vi "Main.vi"() -> ()   [LabVIEW 2026]
uses:
  Typedefs/Test Config.ctl
  Typedefs/Station State.ctl
  Typedefs/Measurement.ctl
  Typedefs/Log Message.ctl
  Typedefs/Log Message Type.ctl
  Typedefs/Chiller Action.ctl
  <vilib>/drjdpowell/SQLite Library/SQL Connection/Connection.lvclass/Connection.ctl
  <vilib>/drjdpowell/SQLite Library/SQL Connection/Execute SQL (No results).vi
  <vilib>/drjdpowell/SQLite Library/SQL Connection/Connection.lvclass
  <vilib>/Analysis/NI_AALPro.lvlib
  <vilib>/drjdpowell/SQLite Library/SQLite.lvlib
panel:
  out "Runs Synced":i32
  out "# elements in queue":i32
  out "Abort Reason":string
  out "Result":string
  out "L-I Curve":cluster{dbl[], dbl[]}(graph)
  out "Power (W)":dbl
  out "Current (A)":dbl
  out "Chiller Temp (C)":dbl
  out "State":T1
  in  "Interlock OK":bool=TRUE
  in  "Quit":bool
  in  "Run Batch":bool
  in  "Abort":bool
  in  "Start":bool
  in  "Test Config":T2={"Setpoint (C)"=25.0, "Serial Number"="LD-0001", "I Start (A)"=0.0, "I Stop (A)"=6.0, "I Step (A)"=0.1, "Ith Max (A)"=0.6, "Slope Min (W/A)"=0.9, "Stabilize Tol (C)"=0.2, "Stabilize Timeout (s)"=300.0, "Over-Temp Limit (C)"=40.0, "Operator"="mahmut", "Fit I Max (A)"=3.0, "Fit P Min (W)"=0.1}
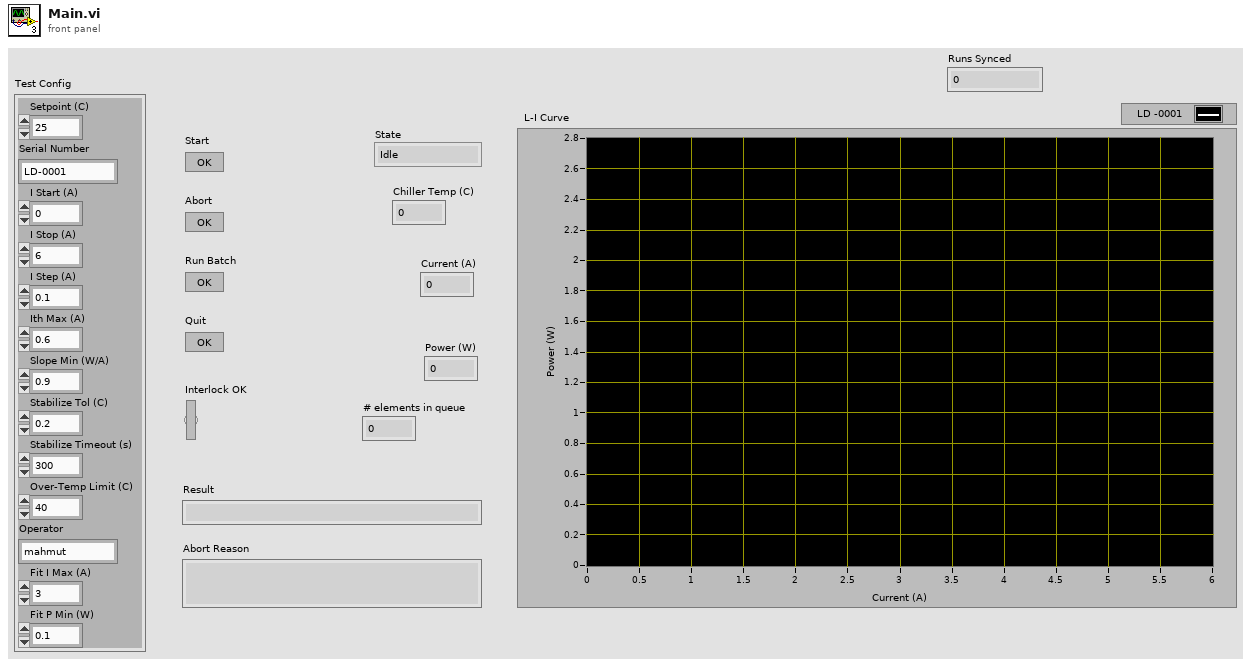
[diagram p1: front panel]
types:
  T1 = typedef "Station State.ctl" = enum16{"Idle", "Initialize", "Chiller Stabilize", "Current Ramp", "Measure", "Evaluate", "Log", "Report", "Safe Shutdown"}
  T2 = typedef "Test Config.ctl" = cluster{"Setpoint (C)":dbl, "Serial Number":string, "I Start (A)":dbl, "I Stop (A)":dbl, "I Step (A)":dbl, "Ith Max (A)":dbl, "Slope Min (W/A)":dbl, "Stabilize Tol (C)":dbl, "Stabilize Timeout (s)":dbl, "Over-Temp Limit (C)":dbl, "Operator":string, "Fit I Max (A)":dbl, "Fit P Min (W)":dbl}
  T3 = typedef "Log Message.ctl" = cluster{"Type":T4, "Serial Number":string, "Measurement":T5, "Pass":bool, "Ith (A)":dbl, "Slope (W/A)":dbl, "Reason":string}
  T4 = typedef "Log Message Type.ctl" = enum16{"Run Start", "Measurement", "Run End", "Stop"}
  T5 = typedef "Measurement.ctl" = cluster{"Current (A)":dbl, "Power (W)":dbl, "Temp (C)":dbl, "t (s)":dbl}
  T6 = enum16{"open", "replace", "create", "open or create", "replace or create", "replace or create with confirmation"}
  T7 = cluster{"Last INSERT RowID":i64, i32, "Current (A)":dbl, "Power (W)":dbl, "Temp (C)":dbl, "t (s)":dbl}
  T8 = cluster{string, "Ith (A)":dbl, "Slope (W/A)":dbl, "Variant":variant, "Reason":string, "Last INSERT RowID":i64}
  T9 = typedef "Chiller Action.ctl" = enum16{"Init", "Set Setpoint", "Step", "Read"}
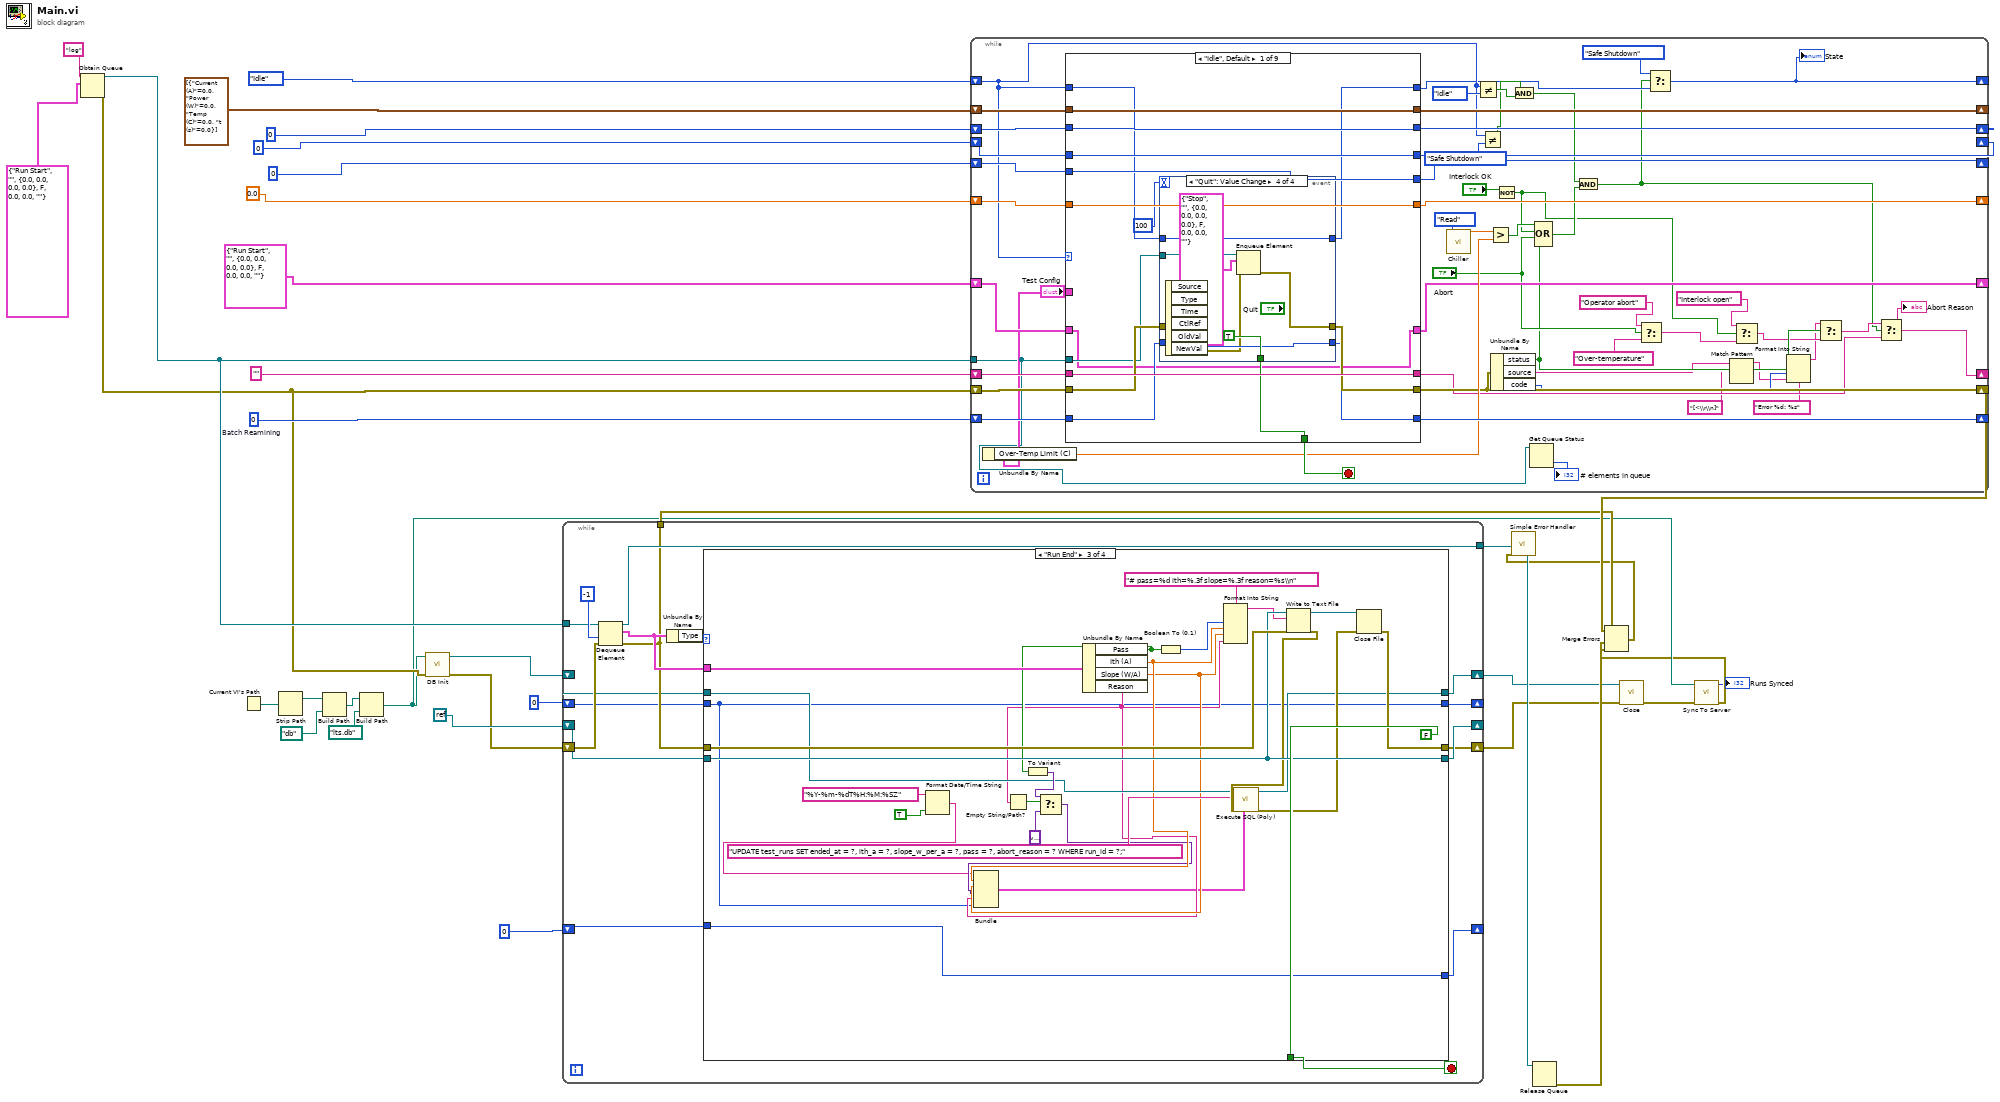
[diagram p0: block diagram]
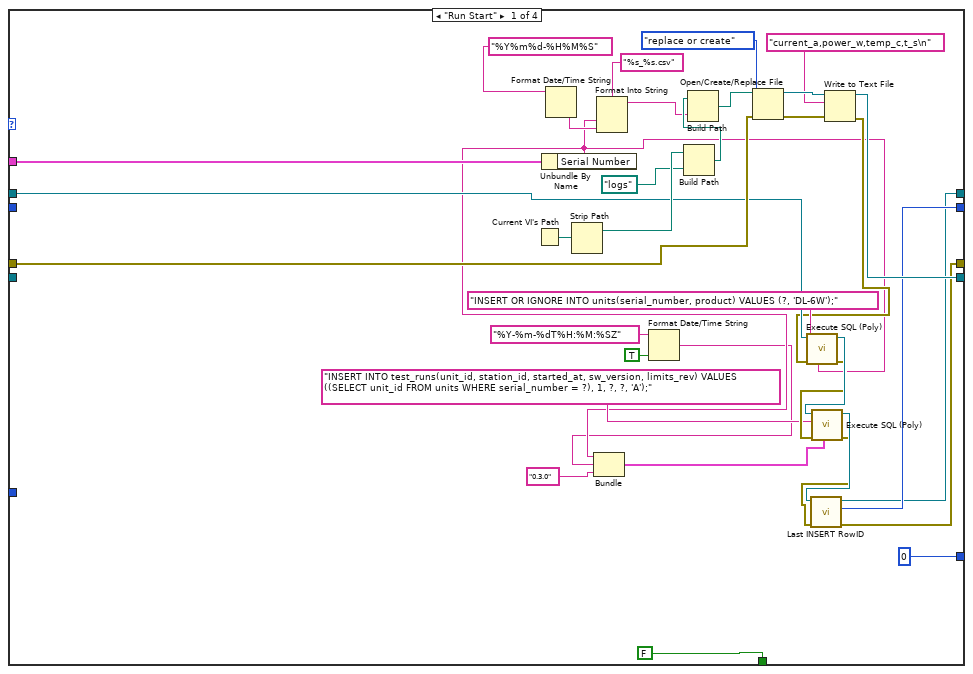
[diagram p2: hidden frame]
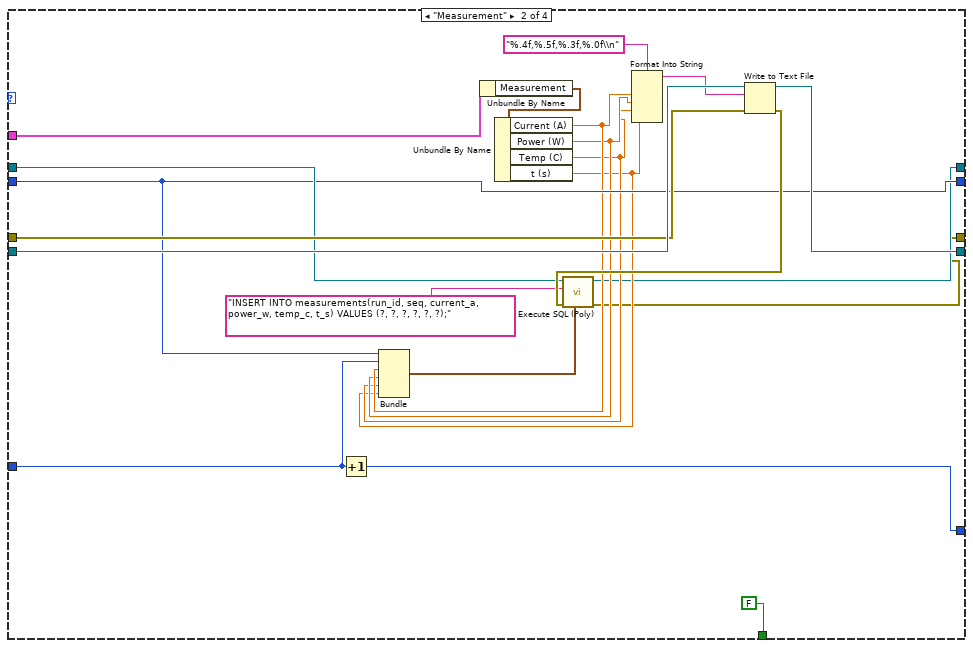
[diagram p3: hidden frame]
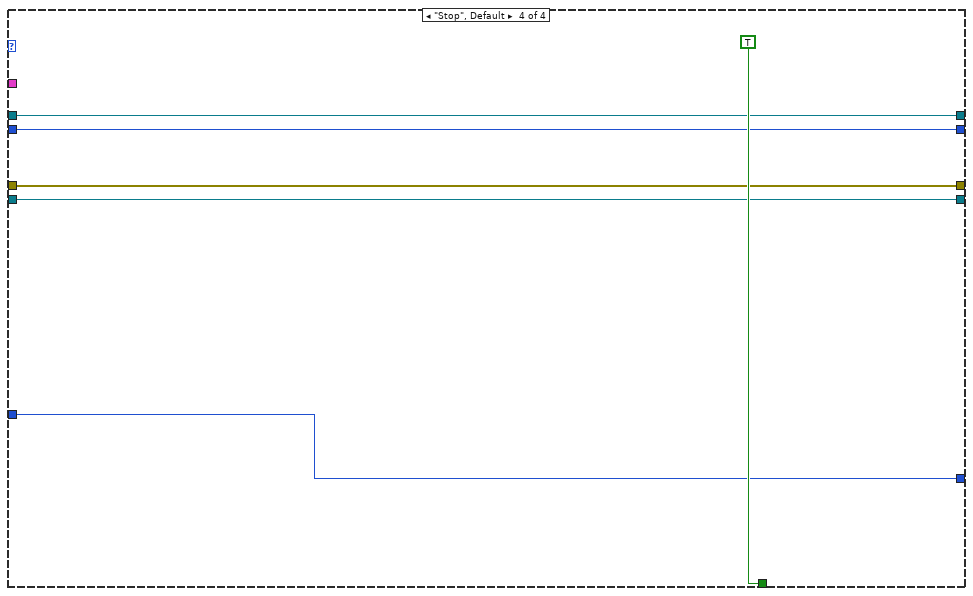
[diagram p4: hidden frame]
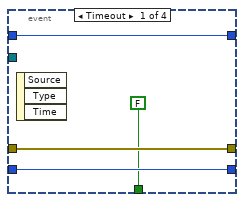
[diagram p5: hidden frame]
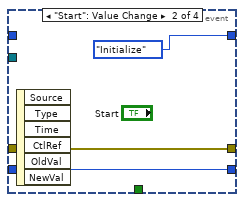
[diagram p6: hidden frame]
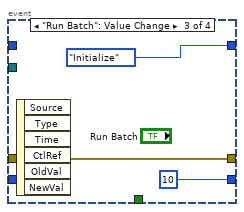
[diagram p7: hidden frame]
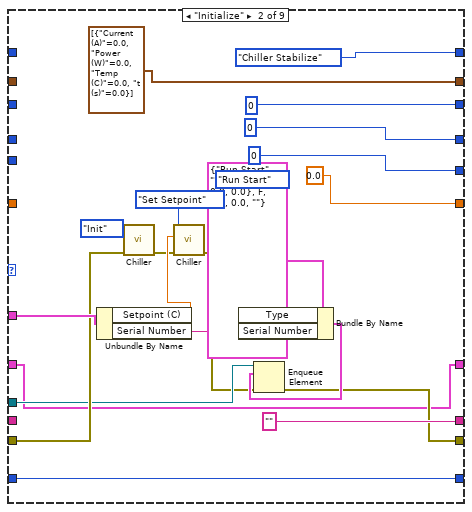
[diagram p8: hidden frame]
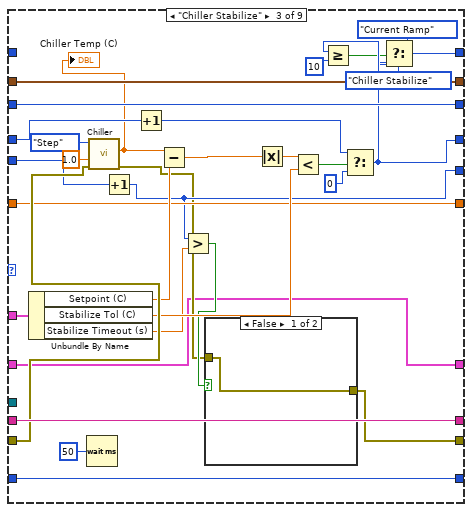
[diagram p9: hidden frame]
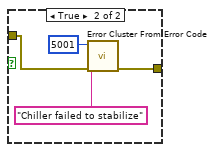
[diagram p10: hidden frame]
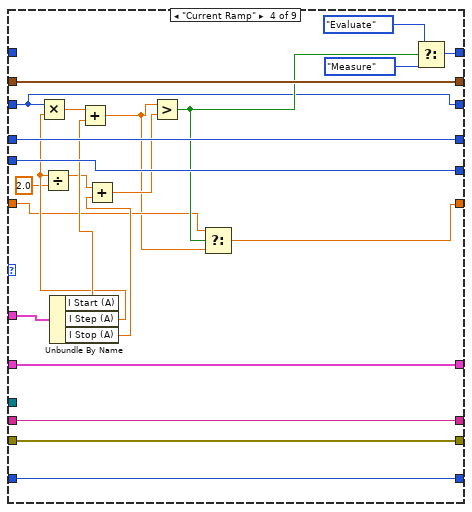
[diagram p11: hidden frame]
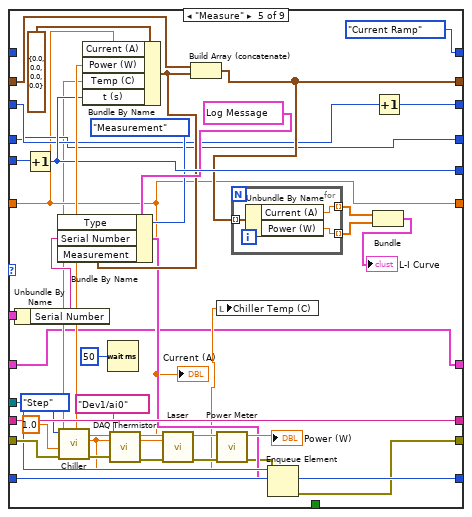
[diagram p12: hidden frame]
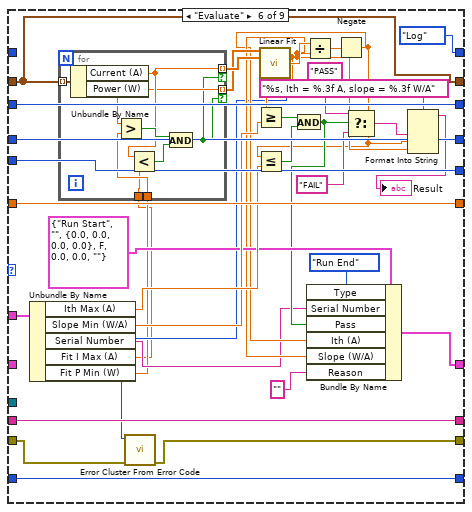
[diagram p13: hidden frame]
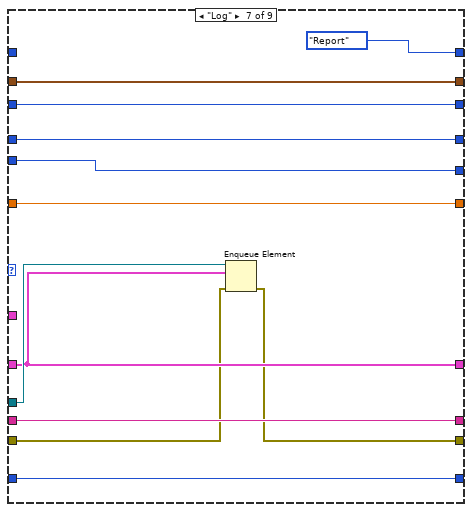
[diagram p14: hidden frame]
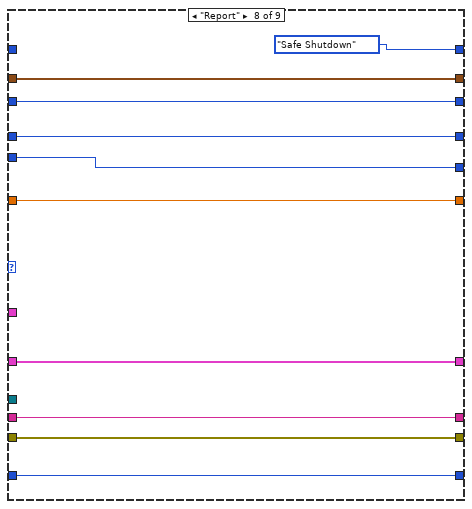
[diagram p15: hidden frame]
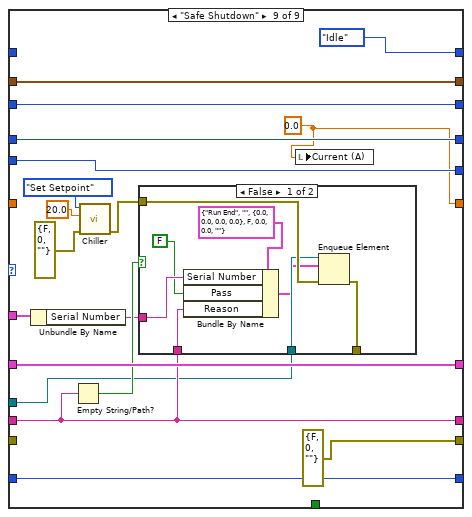
[diagram p16: hidden frame]
diagram:
  w19 = 0  # Batch Reamining
  n1 = Obtain Queue(name (unnamed)="log", element data type=T3 {"Type"=enum."Run Start", "Serial Number"="", "Measurement"={"Current (A)"=0.0, "Power (W)"=0.0, "Temp (C)"=0.0, "t (s)"=0.0}, "Pass"=FALSE, "Ith (A)"=0.0, "Slope (W/A)"=0.0, "Reason"=""} ("Log Message")) -> (queue out=w25:refnum<queue>, error out=w11:errorcluster)  [unwired: 3 in, 1 out]
  n2 = Current VI's Path() -> (path=w16:path)
  n3 = Strip Path(path=w16) -> (stripped path=w15:path)  [unwired: 1 out]
  n4 = Build Path(base path=w15, name or relative path=path "db") -> (appended path=w13:path)
  n5 = Build Path(base path=w13, name or relative path=path "lts.db") -> (appended path=w4:path)
  n6 = call "DB Init.vi"("error in (no error)"=w11, "DB Path"=w4) -> ("error out"=w10:errorcluster, "Connection"=w9:refnum<class "Connection.lvclass">)  [unwired: 8 in]
  n7 = while {
    tunnel: w25 -> [w50]
    tunnel: [w44] -> w23
    tunnel: [w46] -> w21
    shift-right: [w42] -> _
    shift-left: refnum<k0> refnum -> [w43]
    shift-right: [w39] -> w7
    shift-left: w9 -> [w41]
    shift-right: [w37] -> _
    shift-left: i64 0 -> [w40]
    shift-right: [w38] -> w6
    shift-left: w10 -> [w47]
    shift-right: [w35] -> _
    shift-left: 0 -> [w36]
    stop <- w48 stop-if-true
    n8 = Dequeue Element(queue=w50, timeout in ms (-1)=-1, error in (no error)=w47) -> (queue out=w46:refnum<queue>, element=w45:T3, error out=w44:errorcluster)  [unwired: 1 out]
    n9 = Unbundle By Name "Unbundle By Name"(w45) -> ("Type"=w49:T4)
    n10 = case shown="\"Run End\"" w49 {
      tunnel: [FALSE FALSE FALSE TRUE] -> w48
      tunnel: w45 -> [w85 w106 w134 _]
      tunnel: w44 -> [w80 w101 w131 w139]
      tunnel: w43 -> [_ w103 w129 w140]
      tunnel: [w53 w87 w130 w139] -> w38
      tunnel: [w77 w102 w129 w140] -> w42
      tunnel: w41 -> [w69 w97 w118 w138]
      tunnel: [w54 w88 w117 w138] -> w39
      tunnel: w40 -> [_ w95 w108 w137]
      tunnel: [w55 w95 w108 w137] -> w37
      tunnel: w36 -> [_ w94 w111 w136]
      tunnel: [0 w99 w111 w136] -> w35
      frame "Run Start" {
        n11 = Current VI's Path() -> (path=w82:path)
        n12 = Unbundle By Name(w85) -> ("Serial Number"=w61:string)
        n13 = Format Date/Time String(time format string (%c)="%Y%m%d-%H%M%S") -> (date/time string=w75:string)  [unwired: 2 in]
        n14 = Strip Path(path=w82) -> (stripped path=w74:path)  [unwired: 1 out]
        n15 = Format Into String "Format Into String"(format string="%s_%s.csv", w61, w75) -> (resulting string=w71:string)  [unwired: 2 in, 1 out]
        n16 = Format Date/Time String(time format string (%c)="%Y-%m-%dT%H:%M:%SZ", UTC format=TRUE) -> (date/time string=w60:string)  [unwired: 1 in]
        n17 = Bundle("Serial Number"=w61, w60, "0.3.0") -> (w58:cluster{"Serial Number":string, string, string})  [unwired: 1 in]
        n18 = Build Path(base path=w74, name or relative path=path "logs") -> (appended path=w72:path)
        n19 = Build Path(base path=w72, name or relative path=w71) -> (appended path=w81:path)
        n20 = Open/Create/Replace File(file path (use dialog)=w81, error in=w80, operation (0:open)=T6."replace or create") -> (refnum out=w78:refnum<file>, error out=w79:errorcluster)  [unwired: 3 in, 1 out]
        n21 = Write to Text File(file (use dialog)=w78, text="current_a,power_w,temp_c,t_s\n", error in=w79) -> (refnum out=w77:refnum<file>, error out=w67:errorcluster)  [unwired: 1 in, 1 out]
        n22 = call-poly <vilib>:"Execute SQL (Poly).vi"("Parameter(s)"=w61, "error in (no error)"=w67, "SQL"="INSERT OR IGNORE INTO units(serial_number, product) VALUES (?, 'DL-6W');", "SQLite Connection in"=w69) -> ("error out"=w63:errorcluster, "SQLite Connection"=w64:refnum<class "Connection.lvclass">)  [unwired: 6 in]
        n23 = call-poly <vilib>:"Execute SQL (Poly).vi"("Parameter(s)"=w58, "error in (no error)"=w63, "SQL"="INSERT INTO test_runs(unit_id, station_id, started_at, sw_version, limits_rev) VALUES ((SELECT unit_id FROM units WHERE serial_number = ?), 1, ?, ?, 'A');", "SQLite Connection in"=w64) -> ("error out"=w56:errorcluster, "SQLite Connection"=w57:refnum<class "Connection.lvclass">)  [unwired: 6 in]
        n24 = call <vilib>:"Last INSERT RowID.vi"("error in (no error)"=w56, "SQLite Connection in"=w57) -> ("error out"=w53:errorcluster, "Last INSERT RowID"=w55:i64, "SQLite Connection"=w54:refnum<class "Connection.lvclass">)  [unwired: 7 in]
      }
      frame "Measurement" {
        n25 = Increment(x=w94) -> (x+1=w99:i32)
        n26 = Unbundle By Name(w106) -> ("Measurement"=w105:T5)
        n27 = Unbundle By Name(w105) -> ("Current (A)"=w93:dbl, "Power (W)"=w92:dbl, "Temp (C)"=w91:dbl, "t (s)"=w90:dbl)
        n28 = Bundle("Last INSERT RowID"=w95, w94, "Current (A)"=w93, "Power (W)"=w92, "Temp (C)"=w91, "t (s)"=w90) -> (w89:T7)  [unwired: 1 in]
        n29 = Format Into String(format string="%.4f,%.5f,%.3f,%.0f\\n", w93, w92, w91, w90) -> (resulting string=w100:string)  [unwired: 2 in, 1 out]
        n30 = Write to Text File(file (use dialog)=w103, text=w100, error in=w101) -> (refnum out=w102:refnum<file>, error out=w98:errorcluster)  [unwired: 1 in, 1 out]
        n31 = call-poly <vilib>:"Execute SQL (Poly).vi"("Parameter(s)"=w89, "error in (no error)"=w98, "SQL"="INSERT INTO measurements(run_id, seq, current_a, power_w, temp_c, t_s) VALUES (?, ?, ?, ?, ?, ?);", "SQLite Connection in"=w97) -> ("error out"=w87:errorcluster, "SQLite Connection"=w88:refnum<class "Connection.lvclass">)  [unwired: 6 in]
      }
      frame "Run End" {
        n32 = Format Date/Time String(time format string (%c)="%Y-%m-%dT%H:%M:%SZ", UTC format=TRUE) -> (date/time string=w109:string)  [unwired: 1 in]
        n33 = Unbundle By Name(w134) -> ("Pass"=w124:bool, "Ith (A)"=w115:dbl, "Slope (W/A)"=w114:dbl, "Reason"=w112:string)
        n34 = Empty String/Path?(string/path=w112) -> (empty?=w123:bool)
        n35 = To Variant(anything=w124) -> (Variant=w122:variant)
        n36 = Select(t=w122, s=w123, f=variant) -> (s? t:f=w113:variant)
        n37 = Bundle(w109, "Ith (A)"=w115, "Slope (W/A)"=w114, "Variant"=w113, "Reason"=w112, "Last INSERT RowID"=w108) -> (w110:T8)  [unwired: 1 in]
        n38 = Boolean To (0,1)(Boolean=w124) -> (0, 1=w132:i16)
        n39 = Format Into String(format string="# pass=%d ith=%.3f slope=%.3f reason=%s\\n", w132, w115, w114, w112) -> (resulting string=w127:string)  [unwired: 2 in, 1 out]
        n40 = Write to Text File(file (use dialog)=w129, text=w127, error in=w131) -> (refnum out=w128:refnum<file>, error out=w120:errorcluster)  [unwired: 1 in, 1 out]
        n41 = call-poly <vilib>:"Execute SQL (Poly).vi"("Parameter(s)"=w110, "error in (no error)"=w120, "SQL"="UPDATE test_runs SET ended_at = ?, ith_a = ?, slope_w_per_a = ?, pass = ?, abort_reason = ? WHERE run_id = ?;", "SQLite Connection in"=w118) -> ("error out"=w119:errorcluster, "SQLite Connection"=w117:refnum<class "Connection.lvclass">)  [unwired: 6 in]
        n42 = Close File(refnum=w128, error in=w119) -> (error out=w130:errorcluster)  [unwired: 1 out]
      }
      frame "Stop", Default {
      }
    }
  }
  n43 = while {
    shift-right: [w151] -> _
    shift-left: Station_State."Idle" ("Enum") -> [w171]
    shift-right: [w194] -> _
    shift-left: T5[] [{"Current (A)"=0.0, "Power (W)"=0.0, "Temp (C)"=0.0, "t (s)"=0.0}] -> [w195]
    shift-right: [w192] -> _
    shift-left: 0 -> [w193]
    shift-right: [w190] -> _
    shift-left: 0 -> [w191]
    shift-right: [w188] -> _
    shift-left: 0 -> [w189]
    shift-right: [w186] -> _
    shift-left: 0.0 -> [w187]
    shift-right: [w150] -> _
    shift-left: "" -> [w185]
    shift-right: [w175] -> w24
    shift-left: w11 -> [w184]
    tunnel: w25 -> [w149]
    shift-right: [w181] -> _
    shift-left: w19 -> [w182]
    shift-right: [w165] -> _
    shift-left: T3 {"Type"=enum."Run Start", "Serial Number"="", "Measurement"={"Current (A)"=0.0, "Power (W)"=0.0, "Temp (C)"=0.0, "t (s)"=0.0}, "Pass"=FALSE, "Ith (A)"=0.0, "Slope (W/A)"=0.0, "Reason"=""} ("Log Message") -> [w180]
    stop <- w183 stop-if-true
    n44 = Unbundle By Name("Test Config") -> ("Over-Temp Limit (C)"=w177:dbl)
    n45 = case shown="\"Idle\", Default" w171 {
      tunnel: w171 -> [w205 _ _ _ _ _ _ _ _]
      tunnel: [w204 Station_State."Chiller Stabilize" ("Enum") w259 w295 Station_State."Current Ramp" ("Enum") Station_State."Log" ("Enum") Station_State."Report" ("Enum") Station_State."Safe Shutdown" ("Enum") Station_State."Idle" ("Enum")] -> w164
      tunnel: [w211 T5[] [{"Current (A)"=0.0, "Power (W)"=0.0, "Temp (C)"=0.0, "t (s)"=0.0}] w264 w310 w321 w378 w404 w414 w432] -> w194
      tunnel: w195 -> [w211 _ w264 w310 w331 w378 w404 w414 w432]
      tunnel: [w210 0 w282 w289 w316 w384 w403 w413 w431] -> w192
      tunnel: w193 -> [w210 _ w282 w289 w317 w384 w403 w413 w431]
      tunnel: [w209 0 w263 w309 w314 w383 w402 w412 w430] -> w190
      tunnel: w191 -> [w209 _ w270 w309 w314 w383 w402 w412 w430]
      tunnel: [w208 0 w258 w308 w332 w382 w401 w411 w429] -> w188
      tunnel: w189 -> [w208 _ w266 w308 w333 w382 w401 w411 w429]
      tunnel: [w207 0.0 w268 w290 w313 w381 w400 w410 w422] -> w186
      tunnel: w187 -> [w207 _ w268 w292 w313 w381 w400 w410 _]
      tunnel: [w206 "" w281 w307 w346 w356 w399 w409 w416] -> w153
      tunnel: w185 -> [w206 _ w281 w307 w346 w356 w399 w409 w416]
      tunnel: [w202 w230 w253 w306 w322 w353 w393 w408 errorcluster {"status"=FALSE, "code"=0, "source"=""} ("error constant")] -> w175
      tunnel: w184 -> [w203 w244 w276 w306 w344 w354 w394 w408 _]
      tunnel: [w199 _ _ _ _ _ _ _ _] -> w183
      tunnel: w182 -> [w201 w250 w280 w305 w341 w380 w398 w407 w428]
      tunnel: [w200 w250 w280 w305 w341 w380 w398 w407 w428] -> w181
      tunnel: w149 -> [w197 w233 _ _ w325 _ w396 _ w415]
      tunnel: "Test Config" -> [_ w248 w279 w304 w328 w373 _ _ w418]
      tunnel: w180 -> [w196 w229 w251 w288 w311 _ w395 w405 w426]
      tunnel: [w196 w229 w251 w288 w311 w360 w395 w405 w426] -> w165
      frame "Idle", Default {
        n46 = event shown="[3] \"Quit\": Value Change" {
          selector: _ -> [_ _ _ _]
          dyn-events: _ -> [_ _ _ _]
          timeout: 100 -> [_ _ _ _]
          tunnel: w205 -> [w215 _ _ w228]
          tunnel: [w215 Station_State."Initialize" ("Enum") Station_State."Initialize" ("Enum") w228] -> w204
          tunnel: w203 -> [w214 w217 w219 w224]
          tunnel: [w214 w217 w219 w223] -> w202
          tunnel: w201 -> [w213 w218 _ w226]
          tunnel: [w213 w218 10 ("Batch Reamining") w226] -> w200
          tunnel: [FALSE _ _ TRUE] -> w199
          tunnel: w197 -> [_ _ _ w225]
          event Timeout {
            n47 = event-data() -> ()  [unwired: 1 in, 3 out]
          }
          event "Start": Value Change {
            n48 = event-data() -> ()  [unwired: 1 in, 6 out]
          }
          event "Run Batch": Value Change {
            n49 = event-data() -> ()  [unwired: 1 in, 6 out]
          }
          event "Quit": Value Change {
            n50 = event-data() -> ()  [unwired: 1 in, 6 out]
            n51 = Enqueue Element(queue=w225, element=T3 {"Type"=enum."Stop", "Serial Number"="", "Measurement"={"Current (A)"=0.0, "Power (W)"=0.0, "Temp (C)"=0.0, "t (s)"=0.0}, "Pass"=FALSE, "Ith (A)"=0.0, "Slope (W/A)"=0.0, "Reason"=""} ("Log Message"), error in (no error)=w224) -> (error out=w223:errorcluster)  [unwired: 1 in, 2 out]
          }
        }
      }
      frame "Initialize" {
        n52 = Unbundle By Name(w248) -> ("Setpoint (C)"=w245:dbl, "Serial Number"=w234:string)
        n53 = call "Chiller.vi"("error in (no error)"=w244, "Action"=Chiller_Action."Init") -> ("error out"=w243:errorcluster)  [unwired: 5 in, 2 out]
        n54 = call "Chiller.vi"("error in (no error)"=w243, "Setpoint (C)"=w245, "Action"=Chiller_Action."Set Setpoint") -> ("error out"=w231:errorcluster)  [unwired: 4 in, 2 out]
        n55 = Bundle By Name(cluster=T3 {"Type"=enum."Run Start", "Serial Number"="", "Measurement"={"Current (A)"=0.0, "Power (W)"=0.0, "Temp (C)"=0.0, "t (s)"=0.0}, "Pass"=FALSE, "Ith (A)"=0.0, "Slope (W/A)"=0.0, "Reason"=""} ("Log Message"), "Type"=Log_Message_Type."Run Start", "Serial Number"=w234) -> (w232:T3)
        n56 = Enqueue Element(queue=w233, element=w232, error in (no error)=w231) -> (error out=w230:errorcluster)  [unwired: 1 in, 2 out]
      }
      frame "Chiller Stabilize" {
        n57 = Unbundle By Name(w279) -> ("Setpoint (C)"=w275:dbl, "Stabilize Tol (C)"=w272:dbl, "Stabilize Timeout (s)"=w257:dbl)
        n58 = Wait (ms)(milliseconds to wait=u32 50) -> ()  [unwired: 1 out]
        n59 = call "Chiller.vi"("error in (no error)"=w276, "dt (s)"=1.0, "Action"=Chiller_Action."Step") -> ("error out"=w254:errorcluster, "Temp (C)"=w255:dbl)  [unwired: 4 in, 1 out]
        "Chiller Temp (C)" <- w255
        n60 = Increment(x=w266) -> (x+1=w258:i32)
        n61 = Increment(x=w270) -> (x+1=w269:i32)
        n62 = Subtract(x=w255, y=w275) -> (x-y=w274:dbl)
        n63 = Greater?(x=w258, y=w257) -> (0:w256:bool)
        n64 = case shown="False" w256 {
          tunnel: w254 -> [w283 w285]
          tunnel: [w283 w284] -> w253
          frame False {
          }
          frame True {
            n65 = call <vilib>:"Error Cluster From Error Code.vi"("error in (no error)"=w285, "error message (\"\")"="Chiller failed to stabilize" ("error message (\"\")"), "error code (0)"=5001) -> ("error out"=w284:errorcluster)  [unwired: 6 in]
          }
        }
        n66 = Absolute Value(x=w274) -> (abs(x)=w273:dbl)
        n67 = Less?(x=w273, y=w272) -> (x < y?=w271:bool)
        n68 = Select(t=w269, s=w271, f=0) -> (s? t:f=w263:i32)
        n69 = Greater Or Equal?(x=w263, y=10) -> (x >= y?=w262:bool)
        n70 = Select(t=Station_State."Current Ramp" ("Enum"), s=w262, f=Station_State."Chiller Stabilize" ("Enum")) -> (s? t:f=w259:T1)
      }
      frame "Current Ramp" {
        n71 = Unbundle By Name(w304) -> ("I Start (A)"=w302:dbl, "I Step (A)"=w300:dbl, "I Stop (A)"=w301:dbl)
        n72 = Multiply(x=w289, y=w300) -> (x*y=w303:dbl)
        n73 = Divide(x=w300, y=2.0) -> (x/y=w298:dbl)
        n74 = Add(x=w303, y=w302) -> (x+y=w291:dbl)
        n75 = Add(x=w298, y=w301) -> (x+y=w299:dbl)
        n76 = Greater?(x=w291, y=w299) -> (0:w293:bool)
        n77 = Select(t=w292, s=w293, f=w291) -> (s? t:f=w290:dbl)
        n78 = Select(t=Station_State."Evaluate" ("Enum"), s=w293, f=Station_State."Measure" ("Enum")) -> (s? t:f=w295:T1)
      }
      frame "Measure" {
        n79 = Unbundle By Name(w328) -> ("Serial Number"=w327:string)
        n80 = Increment(x=w333) -> (x+1=w332:i32)
        n81 = call "Chiller.vi"("error in (no error)"=w344, "dt (s)"=1.0, "Action"=Chiller_Action."Step") -> ("error out"=w339:errorcluster, "Temp (C)"=w312:dbl)  [unwired: 4 in, 1 out]
        n82 = Wait (ms)(milliseconds to wait=u32 50) -> ()  [unwired: 1 out]
        n83 = call "DAQ Thermistor.vi"("error in (no error)"=w339, "DAQmx Physical Channel"=tag "Dev1/ai0") -> ("error out"=w338:errorcluster)  [unwired: 7 in, 2 out]
        n84 = call "Laser.vi"("error in (no error)"=w338, "Temp (C)"=w312, "Current (A)"=w313) -> ("error out"=w337:errorcluster, "Power (W)"=w336:dbl)  [unwired: 6 in, 1 out]
        n85 = local write "Chiller Temp (C)"(w312) -> ()
        n86 = call "Power Meter.vi"("error in (no error)"=w337, "True Power (W)"=w336) -> ("error out"=w323:errorcluster, "Reading (W)"=w334:dbl)  [unwired: 8 in]
        "Power (W)" <- w334
        n87 = Bundle By Name(cluster=T5 {"Current (A)"=0.0, "Power (W)"=0.0, "Temp (C)"=0.0, "t (s)"=0.0} ("Cluster"), "Current (A)"=w313, "Power (W)"=w334, "Temp (C)"=w312, "t (s)"=w332) -> (w326:T5)
        n88 = Bundle By Name(cluster=T3 {"Type"=enum."Run Start", "Serial Number"="", "Measurement"={"Current (A)"=0.0, "Power (W)"=0.0, "Temp (C)"=0.0, "t (s)"=0.0}, "Pass"=FALSE, "Ith (A)"=0.0, "Slope (W/A)"=0.0, "Reason"=""} ("Log Message"), "Type"=Log_Message_Type."Measurement", "Serial Number"=w327, "Measurement"=w326) -> (w324:T3)
        n89 = Build Array (concatenate)(w331, w326) -> (w321:T5[])
        n90 = for {
          tunnel: w321 -> [w349] mode=indexing
          tunnel: [w348] -> w320 mode=indexing
          tunnel: [w347] -> w319 mode=indexing
          n91 = Unbundle By Name(w349) -> ("Current (A)"=w348:dbl, "Power (W)"=w347:dbl)
        }
        n92 = Enqueue Element(queue=w325, element=w324, error in (no error)=w323) -> (error out=w322:errorcluster)  [unwired: 1 in, 2 out]
        n93 = Bundle(w320, w319) -> (→"L-I Curve":cluster{dbl[], dbl[]})  [unwired: 1 in]
        n94 = Increment(x=w317) -> (x+1=w316:i32)
        "Current (A)" <- w313
      }
      frame "Evaluate" {
        n95 = Unbundle By Name(w373) -> ("Ith Max (A)"=w372:dbl, "Slope Min (W/A)"=w371:dbl, "Serial Number"=w352:string, "Fit I Max (A)"=w350:dbl, "Fit P Min (W)"=w351:dbl)
        n96 = for {
          tunnel: w378 -> [w392] mode=indexing
          tunnel: [w389] -> w377 mode=indexing if=w387
          tunnel: [w388] -> w376 mode=indexing if=w387
          tunnel: w351 -> [w386]
          tunnel: w350 -> [w385]
          n97 = Unbundle By Name(w392) -> ("Current (A)"=w389:dbl, "Power (W)"=w388:dbl)
          n98 = Greater?(x=w388, y=w386) -> (0:w391:bool)
          n99 = Less?(x=w389, y=w385) -> (x < y?=w390:bool)
          n100 = And(x=w391, y=w390) -> (x .and. y?=w387:bool)
        }
        n101 = call <vilib>:"Linear Fit.vi"("Y"=w376, "X"=w377) -> ("slope"=w358:dbl, "intercept"=w375:dbl, "error"=w355:i32)  [unwired: 9 in, 2 out]
        n102 = call <vilib>:"Error Cluster From Error Code.vi"("error in (no error)"=w354, "error code (0)"=w355) -> ("error out"=w353:errorcluster)  [unwired: 7 in]
        n103 = Greater Or Equal?(x=w358, y=w371) -> (x >= y?=w370:bool)
        n104 = Divide(x=w375, y=w358) -> (x/y=w374:dbl)
        n105 = Negate(x=w374) -> (-x=w357:dbl)
        n106 = Less Or Equal?(x=w357, y=w372) -> (x <= y?=w369:bool)
        n107 = And(x=w370, y=w369) -> (x .and. y?=w359:bool)
        n108 = Bundle By Name(cluster=T3 {"Type"=enum."Run Start", "Serial Number"="", "Measurement"={"Current (A)"=0.0, "Power (W)"=0.0, "Temp (C)"=0.0, "t (s)"=0.0}, "Pass"=FALSE, "Ith (A)"=0.0, "Slope (W/A)"=0.0, "Reason"=""} ("Log Message"), "Type"=Log_Message_Type."Run End", "Serial Number"=w352, "Pass"=w359, "Ith (A)"=w357, "Slope (W/A)"=w358, "Reason"="") -> (w360:T3)
        n109 = Select(t="PASS", s=w359, f="FAIL") -> (s? t:f=w365:string)
        n110 = Format Into String(format string="%s, Ith = %.3f A, slope = %.3f W/A", w365, w357, w358) -> (resulting string=→"Result":string)  [unwired: 2 in, 1 out]
      }
      frame "Log" {
        n111 = Enqueue Element(queue=w396, element=w395, error in (no error)=w394) -> (error out=w393:errorcluster)  [unwired: 1 in, 2 out]
      }
      frame "Report" {
      }
      frame "Safe Shutdown" {
        w422 = 0.0
        n112 = Unbundle By Name(w418) -> ("Serial Number"=w417:string)
        n113 = Empty String/Path?(string/path=w416) -> (empty?=w421:bool)
        n114 = call "Chiller.vi"("error in (no error)"=errorcluster {"status"=FALSE, "code"=0, "source"=""} ("error constant"), "Setpoint (C)"=20.0, "Action"=Chiller_Action."Set Setpoint") -> ("error out"=w420:errorcluster)  [unwired: 4 in, 2 out]
        n115 = case shown="False" w421 {
          tunnel: w420 -> [w439 w441]
          tunnel: [w438 w441] -> _
          tunnel: w417 -> [w437 _]
          tunnel: w416 -> [w435 _]
          tunnel: w415 -> [w434 _]
          frame False {
            n116 = Bundle By Name(cluster=T3 {"Type"=enum."Run End", "Serial Number"="", "Measurement"={"Current (A)"=0.0, "Power (W)"=0.0, "Temp (C)"=0.0, "t (s)"=0.0}, "Pass"=FALSE, "Ith (A)"=0.0, "Slope (W/A)"=0.0, "Reason"=""} ("Log Message"), "Serial Number"=w437, "Pass"=FALSE, "Reason"=w435) -> (w433:T3)
            n117 = Enqueue Element(queue=w434, element=w433, error in (no error)=w439) -> (error out=w438:errorcluster)  [unwired: 1 in, 2 out]
          }
          frame True {
          }
        }
        n118 = local write "Current (A)"(w422) -> ()
      }
    }
    n119 = call "Chiller.vi"("Action"=Chiller_Action."Read") -> ("Temp (C)"=w176:dbl)  [unwired: 6 in, 2 out]
    n120 = Not Equal?(x=w171, y=Station_State."Idle") -> (x != y?=w169:bool)
    n121 = Not Equal?(x=w171, y=Station_State."Safe Shutdown") -> (x != y?=w168:bool)
    n122 = Greater?(x=w176, y=w177) -> (0:w173:bool)
    n123 = Unbundle By Name(w175) -> ("status"=w157:bool, "source"=w147:string, "code"=w144:i32)
    n124 = Not(x="Interlock OK") -> (.not. x?=w152:bool)
    n125 = And(x=w168, y=w169) -> (x .and. y?=w167:bool)
    n126 = Get Queue Status(queue=w149) -> (# elements in queue=→"# elements in queue":i32)  [unwired: 2 in, 7 out]
    n127 = Compound Arithmetic op=OR(w173, w152, "Abort", w157) -> (w166:bool)
    n128 = And(x=w167, y=w166) -> (x .and. y?=w154:bool)
    n129 = Select(t="Operator abort", s="Abort", f="Over-temperature") -> (s? t:f=w158:string)
    n130 = Select(t=Station_State."Safe Shutdown", s=w154, f=w164) -> (s? t:f=w151:T1)
    "State" <- w151
    n131 = Match Pattern(string=w147, regular expression="[<\\r\\n]") -> (before substring=w143:string)  [unwired: 1 in, 3 out]
    n132 = Select(t="Interlock open", s=w152, f=w158) -> (s? t:f=w156:string)
    n133 = Format Into String(format string="Error %d: %s", w144, w143) -> (resulting string=w142:string)  [unwired: 2 in, 1 out]
    n134 = Select(t=w142, s=w157, f=w156) -> (s? t:f=w155:string)
    n135 = Select(t=w155, s=w154, f=w153) -> (s? t:f=w150:string)
    "Abort Reason" <- w150
  }
  n136 = Release Queue(queue=w21) -> (error out=w22:errorcluster)  [unwired: 2 in, 2 out]
  n137 = call-dynamic "Close.vi"("error in (no error)"=w6, "SQLite Connection in"=w7) -> ("error out"=w3:errorcluster)  [unwired: 9 in]
  n138 = call "Sync To Server.vi"("error in (no error)"=w3, "DB Path"=w4) -> ("error out"=w2:errorcluster, "Runs Synced"=→"Runs Synced":i32)  [unwired: 8 in]
  n139 = Merge Errors(w24, w23, w22, w2) -> (w20:errorcluster)
  n140 = call <vilib>:"Simple Error Handler.vi"("error in (no error)"=w20) -> ()  [unwired: 4 in, 5 out]
